vi "UNO Q connect.vi"(4 "error in":errorcluster, 6 "port":u32, 7 "Base URL":string) -> (0 "error out":errorcluster, 3 "Session out":T1={"HTTP client"=refnum, "Base URL"="", "Connected"=TRUE})   [LabVIEW 2021]
uses:
  UNO Q Session.ctl
  <vilib>/httpClient/ClientHandle.ctl
  <vilib>/httpClient/POSTBuffer.vi
  <vilib>/httpClient/LabVIEWHTTPClient.lvlib
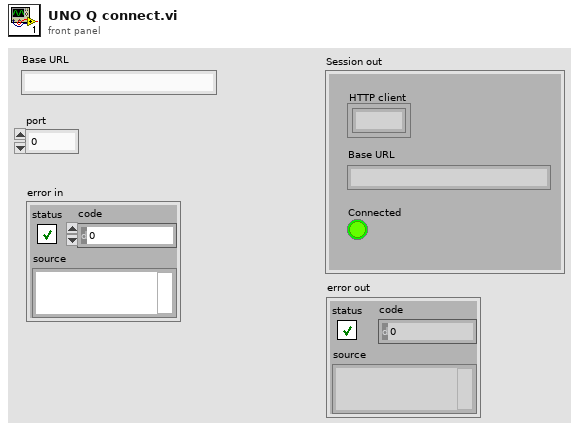
[diagram p1: front panel]
types:
  T1 = typedef "UNO Q Session.ctl" = cluster{"HTTP client":T2, "Base URL":string, "Connected":bool}
  T2 = typedef "LabVIEWHTTPClient.lvlib/ClientHandle.ctl" = refnum<k1>
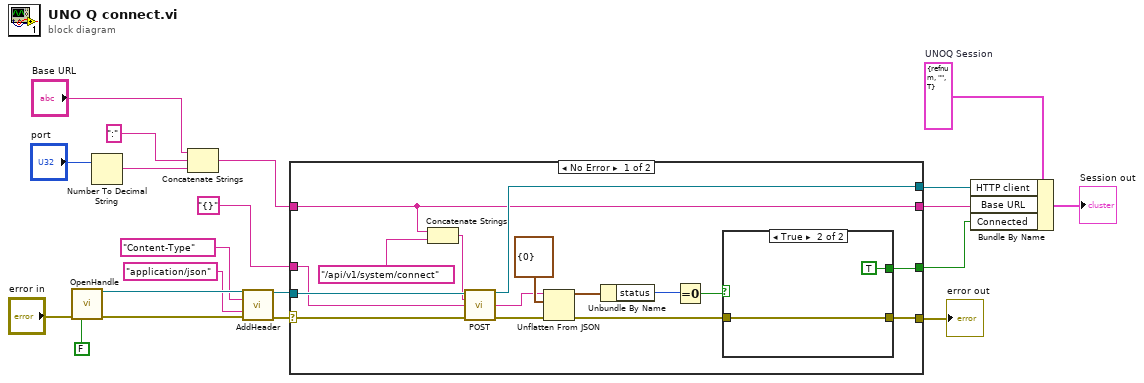
[diagram p0: block diagram]
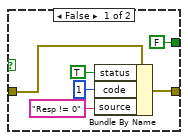
[diagram p2: hidden frame]
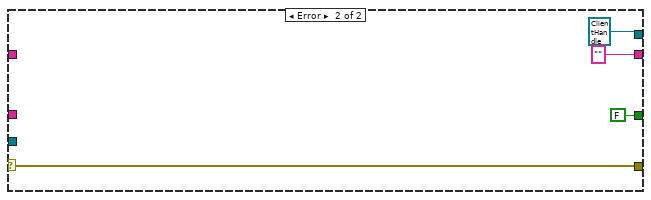
[diagram p3: hidden frame]
diagram:
  w5 = T1 {"HTTP client"=refnum, "Base URL"="", "Connected"=TRUE}  # UNOQ Session
  n1 = call <vilib>:"OpenHandle.vi"("error in (no error)"="error in", "verify server(true)"=FALSE) -> ("client handle out"=w20:T2, "error out"=w16:errorcluster)  [unwired: 12 in]
  n2 = Number To Decimal String(number="port") -> (decimal integer string=w14:string)  [unwired: 1 in]
  n3 = Concatenate Strings("Base URL", ":" ("string"), w14) -> (w10:string)
  n4 = call <vilib>:"AddHeader.vi"("client handle"=w20, "header"="Content-Type", "value"="application/json", "error in (no error)"=w16) -> ("client handle out"=w11:T2, "error out"=w8:errorcluster)  [unwired: 10 in]
  n5 = case shown="No Error" w8 {
    selector: w8 -> [w34 w48]
    tunnel: w11 -> [w36 _]
    tunnel: w10 -> [w22 _]
    tunnel: "{}" ("buffer") -> [w35 _]
    tunnel: [w30 w48] -> w7
    tunnel: [w22 "" ("body")] -> w3
    tunnel: [w25 T2 refnum ("client handle out")] -> w4
    tunnel: [w24 FALSE] -> w2
    frame No Error {
      n6 = Concatenate Strings(w22, "/api/v1/system/connect" ("string")) -> (w23:string)
      n7 = call-poly <vilib>:"POST.vi"("client handle"=w36, "url"=w23, "buffer"=w35, "error in (no error)"=w34) -> ("client handle out"=w25:T2, "body"=w26:string, "error out"=w33:errorcluster)  [unwired: 8 in, 1 out]
      n8 = Unflatten From JSON(JSON string=w26, type and defaults=cluster{"status":i32} {"status"=0}, error in (no error)=w33) -> (value=w28:cluster{"status":i32}, error out=w31:errorcluster)  [unwired: 4 in]
      n9 = Unbundle By Name(w28) -> ("status"=w27:i32)
      n10 = Equal To 0?(x=w27) -> (x = 0?=w32:bool)
      n11 = case shown="True" w32 {
        tunnel: w31 -> [w42 w44]
        tunnel: [w41 w44] -> w30
        tunnel: [FALSE TRUE] -> w24
        frame False {
          n12 = Bundle By Name(cluster=w42, "status"=TRUE, "code"=1, "source"="Resp != 0") -> (w41:errorcluster)
        }
        frame True {
        }
      }
    }
    frame Error {
    }
  }
  "error out" <- w7
  n13 = Bundle By Name(cluster=w5, "HTTP client"=w4, "Base URL"=w3, "Connected"=w2) -> (→"Session out":T1)
